vi "CSM-Logger-Thread.vi"(4 "Log Limit":T1={"file size (in bytes)"=10000000, "file num"=2} {"file size (in bytes)" format="%.0p"}, 6 "Exit When All Module Exist? (F)":bool, 7 "Format String":string="%<%Y/%m/%d %H:%M:%S%3u>T", 8 "error in (no error)":errorcluster, 9 "WatchDogQ":refnum<queue>, 10 "GlobalLogFilter.lvclass":refnum<class "LogFilter.lvclass">, 11 "File Path (Use Dialog)":path) -> (0 "error out":errorcluster)   [LabVIEW 2017, in "CSM File Logger.lvlib"]
doc: "The thread VI used in the CSM - Start File Logger VI.\n\n\n> [!NOTE] <b>CSM File Logger Implementation Principle</b>\n>\n> The CSM File Logger retrieves all execution records in the application via the CSM Global Log API and saves them to a specified text file for later analysis and error localization. The file format is a text file with the suffix `.csmlog`, which can be opened using text editing query tools such as Notepad."
uses:
  CSM File Logger.lvlib
  _Support/GlobalEvent/LogFilter/LogFilter.lvclass
  Communicable State Machine.lvlib
  _Support/Typedef/_CSM_List Module Scope.ctl
  _Shared/CSM Shared.lvlib
  CSM File Logger Limit.ctl
panel:
  in  "internal Stop":bool
  out "#MsgInQueue":i32
  out "size (in bytes)":i64
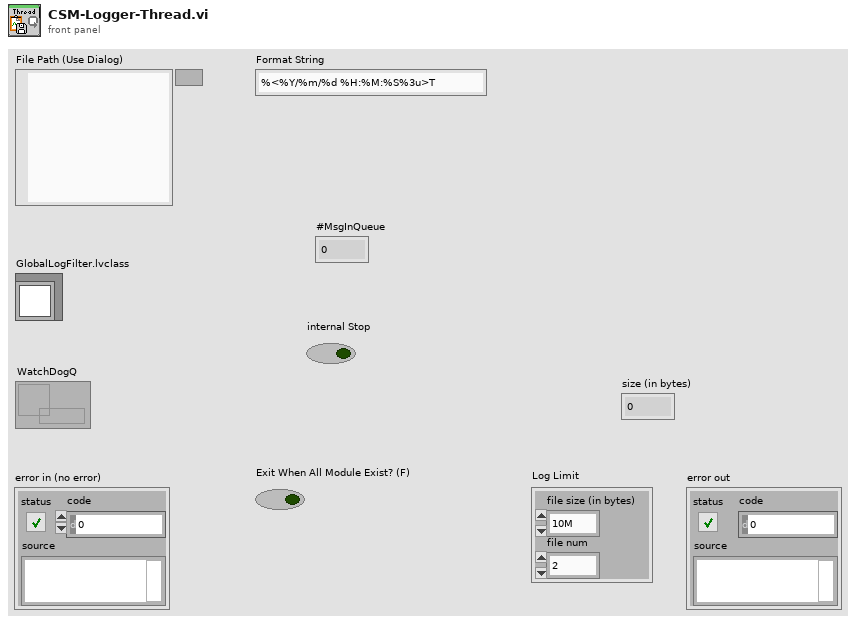
[diagram p1: front panel]
types:
  T1 = typedef "CSM File Logger.lvlib/CSM File Logger Limit.ctl" = cluster{"file size (in bytes)":i64, "file num":i32}
  T2 = typedef "Communicable State Machine.lvlib/_CSM_GlobalLog Filter Rules - v1.2.ctl" = cluster{"Global":cluster{"CSM":string[], "LogType":T3[], "State":string[], "StateType":T4[], "Broadcast":string[]}, "CSM":cluster{"LogType":cluster{"CSM":string, "LogType":T3}[], "State":cluster{"CSM":string, "State":string}[], "StateType":cluster{"CSM":string, "LogType":T4}[], "Broadcast":cluster{"CSM":string, "Broadcast":string}[]}, "PeriodicMessageFilter":cluster{"Enable":bool, "Threshold(#/s)":dbl, "CheckPeriod(s)":dbl}}
  T3 = typedef "Communicable State Machine.lvlib/_CSM_GlobalLog_MSG_TYPE.ctl" = enum16{"User Log", "State Change", "Status", "Interrupt", "Register", "Unregister", "Error Log", "Module Created", "Module Destroyed", "Async Message", "No-Rep Async Message", "Sync Message", "AsyncMsg Complete", "SyncMsg Complete"}
  T4 = typedef "Communicable State Machine.lvlib/_CSM_GlobalLog_STATE_TYPE.ctl" = enum16{"State - Internal State", "State - External Message", "State - Response", "State - Complete"}
  T5 = cluster{"Queue":path[], "folder":path, "name":string, "index":i32, "Log Limit":T1}
  T6 = enum16{"open", "replace", "create", "open or create", "replace or create", "replace or create with confirmation"}
  T7 = typedef "Communicable State Machine.lvlib/_CSM_List Module Scope.ctl" = enum16{"Normal", "System Only", "All"}
  T8 = typedef "Communicable State Machine.lvlib/Periodic String Filter Level.ctl" = enum16{"normal", "L1", "L2", "L3", "L4"}
  T9 = typedef "Communicable State Machine.lvlib/_CSM_GlobalLog_MSG.ctl" = cluster{"Name (\"\" to Use UUID)":string, "Current State":string, "Arguments":string, "Source Message":T10, "Source Module":string, "Complete(T)/Start(F)":bool, "LogType":T3, "Time Stamp":timestamp}
  T10 = typedef "Communicable State Machine.lvlib/_CSM_Response Source Message.ctl" = cluster{"‘State":string, "’Arguments":string, "’Error":errorcluster}
  T11 = cluster{"Major":u16, "Minor":u16, "Fix":u16, "Build":u16}
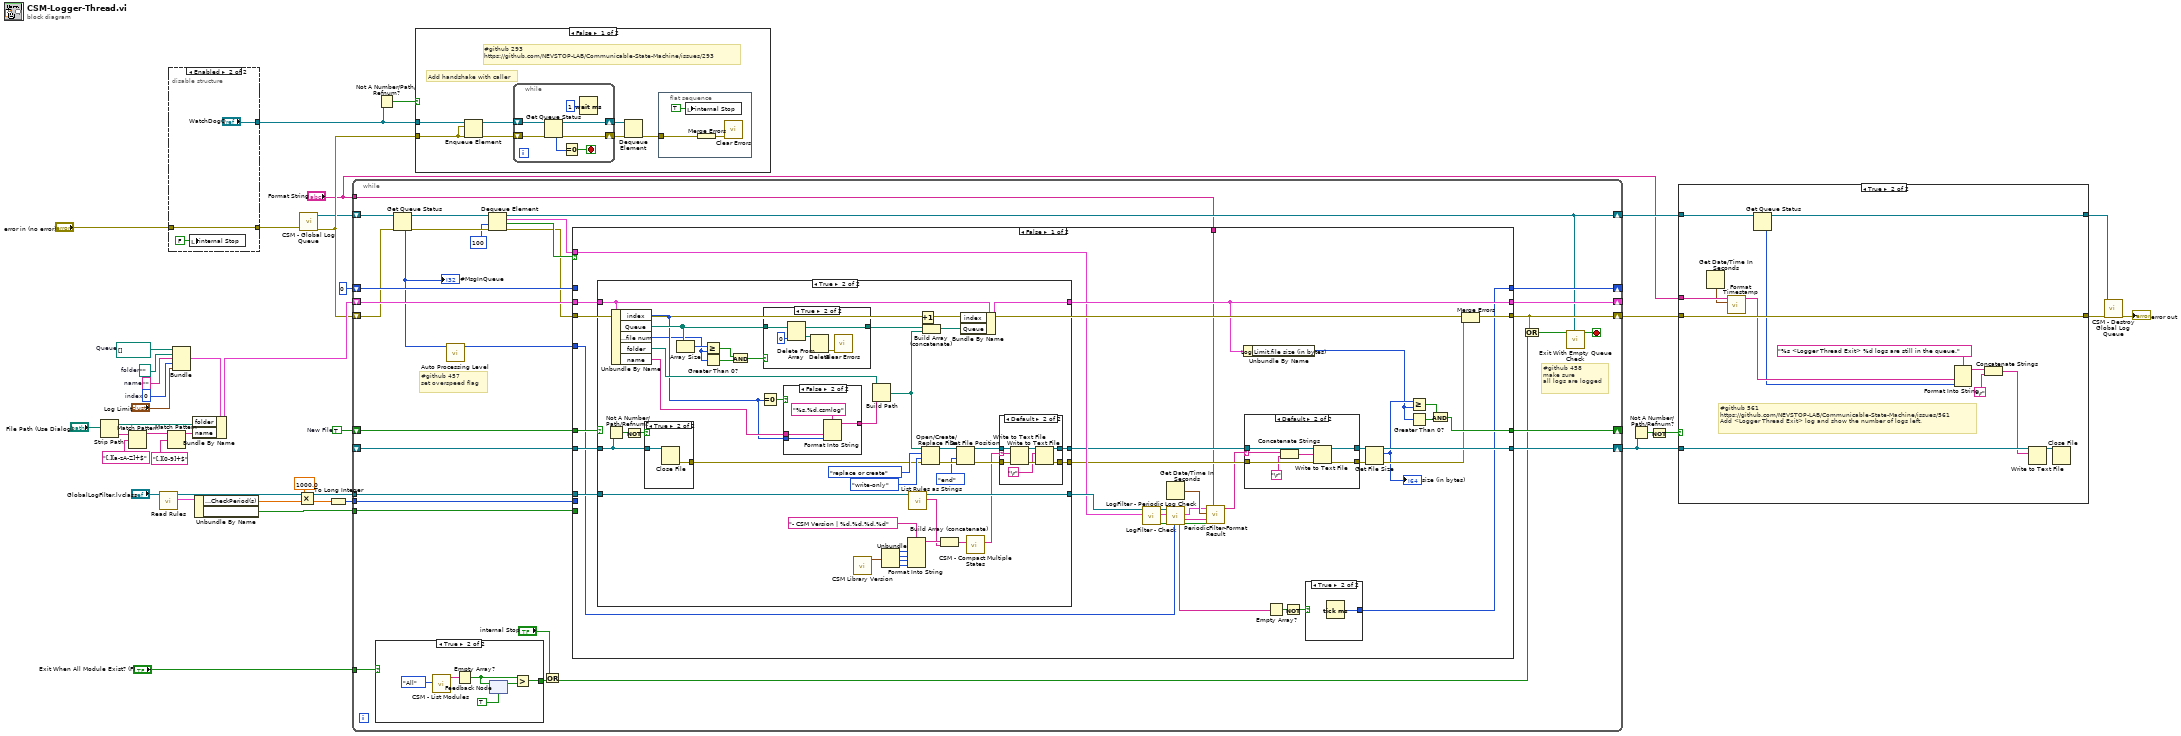
[diagram p0: block diagram]
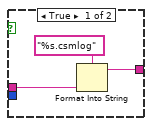
[diagram p6: hidden frame]
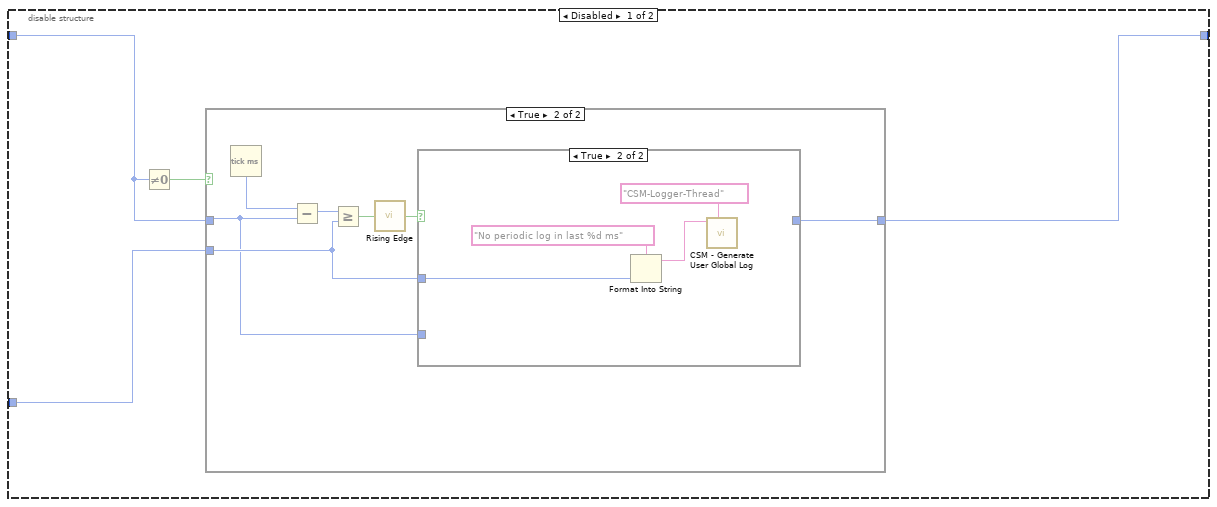
[diagram p10: hidden frame]
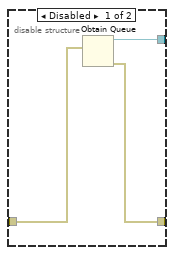
[diagram p15: hidden frame]
diagram:
  w28 = ""  # name
  w31 = 0  # index
  w32 = path ""  # folder
  w33 = path[] []  # Queue
  w34 = TRUE  # New File
  n1 = Strip Path(path="File Path (Use Dialog)") -> (stripped path=w21:path, name=w27:string)
  n2 = Match Pattern(string=w27, regular expression="[.][a-zA-Z]+$") -> (before substring=w24:string)  [unwired: 1 in, 3 out]
  n3 = call "Read Rules.vi"("LogFilter In"="GlobalLogFilter.lvclass") -> ("Rules"=w16:T2, "LogFilter Out"=w17:refnum<class "LogFilter.lvclass">)  [unwired: 8 in, 1 out]
  n4 = Match Pattern(string=w24, regular expression="[.][0-9]+$") -> (before substring=w22:string)  [unwired: 1 in, 3 out]
  n5 = disable-structure shown="Enabled" {
    disable-tunnel: [w41 "WatchDogQ"] -> w40
    disable-tunnel: [w43 w45] -> w6
    disable-tunnel: "error in (no error)" -> [w42 w45]
    frame Disabled {
      n6 = Obtain Queue(element data type=w42) -> (queue out=w41:refnum<queue>, error out=w43:errorcluster)  [unwired: 4 in, 1 out]
    }
    frame Enabled {
      n7 = local write "internal Stop"(FALSE ("internal Stop")) -> ()
    }
  }
  n8 = Bundle("Queue"=w33, "folder"=w32, "name"=w28, "index"=w31, "Log Limit"="Log Limit") -> (w29:T5)  [unwired: 1 in]
  n9 = Bundle By Name(cluster=w29, "folder"=w21, "name"=w22) -> (w23:T5)
  n10 = Unbundle By Name(w16) -> ("PeriodicMessageFilter.CheckPeriod(s)"=w14:dbl, "PeriodicMessageFilter.Enable"=w15:bool)
  n11 = Multiply(x=1000.0, y=w14) -> (x*y=w13:dbl)
  n12 = call "CSM - Global Log Queue.vi"("Error In"=w6) -> ("error out"=w9:errorcluster, "Global Log Queue"=w7:refnum<queue>)  [unwired: 9 in]
  n13 = To Long Integer(number=w13) -> (32bit integer=w11:i32)
  n14 = while {
    shift-right: [w76] -> w4
    shift-left: w9 -> [w59]
    shift-right: [w74] -> w36
    shift-left: _ -> [w75]
    tunnel: "Exit When All Module Exist? (F)" -> [w58]
    shift-right: [w72] -> _
    shift-left: w34 -> [w73]
    shift-right: [w70] -> _
    shift-left: w23 -> [w71]
    tunnel: w17 -> [w69]
    tunnel: w15 -> [w66]
    tunnel: w11 -> [w68]
    shift-right: [w67] -> _
    shift-left: u32 0 ("millisecond timer value") -> [w65]
    shift-right: [w50] -> w2
    shift-left: w7 -> [w62]
    tunnel: "Format String" -> [w47]
    stop <- w51 stop-if-true
    # "#github 458\nmake sure \nall logs are logged"
    # "#github 457\nset overspeed flag"
    n15 = case shown="True" w58 {
      tunnel: [_ w216] -> w57
      frame False {
      }
      frame True {
        n16 = call "CSM - List Modules.vi"("Scope (Normal)"=_CSM_List_Module_Scope."All" ("Mode")) -> ("Module Names"=w220:string[])  [unwired: 9 in, 1 out]
        n17 = Empty Array?(array=w220) -> (empty?=w219:bool)
        n18 = feedback #1(TRUE ("All?")) -> (w218:bool)
        n19 = feedback-in #1(w219) -> ()
        n20 = Greater?(x=w219, y=w218) -> (0:w216:bool)
      }
    }
    n21 = Get Queue Status(queue=w62, error in (no error)=w59) -> (queue out=w61:refnum<queue>, error out=w60:errorcluster, # elements in queue=w49:i32)  [unwired: 1 in, 5 out]
    "#MsgInQueue" <- w49
    n22 = call "Auto Processing Level.vi"("#Left In Q"=w49) -> ("Level"=w48:T8)  [unwired: 8 in, 2 out]
    n23 = Dequeue Element(queue=w61, timeout in ms (-1)=100, error in (no error)=w60) -> (queue out=w50:refnum<queue>, element=w53:T9, timed out?=w64:bool, error out=w63:errorcluster)
    n24 = Or(x="internal Stop", y=w57) -> (x .or. y?=w55:bool)
    n25 = case shown="False" w64 {
      tunnel: w63 -> [w110 w197]
      tunnel: [w109 w197] -> w76
      tunnel: w75 -> [w108 w196]
      tunnel: [w107 w196] -> w74
      tunnel: w73 -> [w106 w195]
      tunnel: [w105 w195] -> w72
      tunnel: w71 -> [w104 w194]
      tunnel: [w103 w194] -> w70
      tunnel: w69 -> [w102 _]
      tunnel: w68 -> [_ w193]
      tunnel: [w101 w191] -> w67
      tunnel: w66 -> [_ _]
      tunnel: w65 -> [_ w192]
      tunnel: w53 -> [w91 _]
      tunnel: w48 -> [w86 _]
      tunnel: w47 -> [w77 _]
      frame False {
        n26 = case shown="True" w106 {
          tunnel: w108 -> [w123 w163]
          tunnel: [_ w135] -> w88
          tunnel: [w123 w136] -> w87
          tunnel: [w122 w152] -> w103
          tunnel: w104 -> [w122 w154]
          tunnel: [w121 w134] -> w95
          tunnel: w102 -> [w121 w139]
          frame False {
          }
          frame True {
            n27 = Not A Number/Path/Refnum?(number/path/refnum=w163) -> (NaN/Path/Refnum?=w164:bool)
            n28 = Unbundle By Name(w154) -> ("index"=w144:i32, "Queue"=w155:path[], "Log Limit.file num"=w141:i32, "folder"=w148:path, "name"=w147:string)
            n29 = Not(x=w164) -> (.not. x?=w165:bool)
            n30 = case shown="True" w165 {
              tunnel: w163 -> [_ w190]
              tunnel: [_ w189] -> w157
              frame False {
              }
              frame True {
                n31 = Close File(refnum=w190) -> (error out=w189:errorcluster)  [unwired: 1 in, 1 out]
              }
            }
            n32 = Array Size(array=w155) -> (size(s)=w156:i32)
            n33 = Greater Or Equal?(x=w156, y=w141) -> (x >= y?=w143:bool)
            n34 = Greater Than 0?(x=w141) -> (x > 0?=w142:bool)
            n35 = And(x=w143, y=w142) -> (x .and. y?=w140:bool)
            n36 = Equal To 0?(x=w144) -> (x = 0?=w145:bool)
            n37 = case shown="True" w140 {
              tunnel: w155 -> [w183 w188]
              tunnel: [w183 w184] -> w153
              frame False {
              }
              frame True {
                n38 = Delete From Array(array=w188, index=0) -> (deleted portion=w186:path, array with subset deleted=w184:path[])  [unwired: 1 in]
                n39 = Delete(path (use dialog)=w186) -> (error out=w185:errorcluster)  [unwired: 4 in, 2 out]
                n40 = call <vilib>:"Clear Errors.vi"("error in (no error)"=w185) -> ()  [unwired: 5 in, 2 out]
              }
            }
            n41 = case shown="False" w145 {
              tunnel: [w177 w181] -> w149
              tunnel: w147 -> [w176 w180]
              tunnel: w144 -> [_ w179]
              frame True {
                n42 = Format Into String(format string="%s.csmlog", w176) -> (resulting string=w177:string)  [unwired: 2 in, 1 out]
              }
              frame False {
                n43 = Format Into String(format string="%s.%d.csmlog", w180, w179) -> (resulting string=w181:string)  [unwired: 2 in, 1 out]
              }
            }
            n44 = call "CSM Library Version.vi"() -> ("Min-Compatible Version"=w132:T11)  [unwired: 10 in, 1 out]
            n45 = Build Path(base path=w148, name or relative path=w149) -> (appended path=w146:path)
            n46 = Unbundle(w132) -> ("Major"=w128:u16, "Minor"=w129:u16, "Fix"=w130:u16, "Build"=w131:u16)
            n47 = Format Into String(format string="- CSM Version | %d.%d.%d.%d" ("String to Prepend to Source (\"\")"), w128, w129, w130, w131) -> (resulting string=w126:string)  [unwired: 2 in, 1 out]
            n48 = call "List Rules as Strings.vi"("GlobalLogFilter In"=w139) -> ("Rule Strings"=w125:string[], "GlobalLogFilter Out"=w134:refnum<class "LogFilter.lvclass">)  [unwired: 8 in, 1 out]
            n49 = Increment(x=w144) -> (x+1=w150:i32)
            n50 = Open/Create/Replace File(file path (use dialog)=w146, error in=w157, operation (0:open)=T6."replace or create", access (0:read/write)=enum16{"read/write", "read-only", "write-only"}."write-only") -> (refnum out=w162:refnum<file>, error out=w161:errorcluster)  [unwired: 2 in, 1 out]
            n51 = Build Array (concatenate)(w153, w146) -> (w151:path[])
            n52 = Build Array (concatenate)(w126, w125) -> (w124:string[])
            n53 = Set File Position(refnum=w162, from (0:start)=enum16{"start", "end", "current"}."end", error in=w161) -> (refnum out=w137:refnum<file>, error out=w138:errorcluster)  [unwired: 1 in]
            n54 = Bundle By Name(cluster=w154, "index"=w150, "Queue"=w151) -> (w152:T5)
            n55 = call "CSM - Compact Multiple States.vi"("Multiple States"=w124) -> ("States"=w133:string)  [unwired: 9 in]
            n56 = case shown="Default" w133 {
              selector: w133 -> [_ w175]
              tunnel: w138 -> [w166 w174]
              tunnel: w137 -> [w167 w173]
              tunnel: [w167 w170] -> w136
              tunnel: [w166 w169] -> w135
              frame "" {
              }
              frame Default {
                n57 = Write to Text File(file (use dialog)=w173, text=w175, error in=w174) -> (refnum out=w171:refnum<file>, error out=w172:errorcluster)  [unwired: 1 in, 1 out]
                n58 = Write to Text File(file (use dialog)=w171, text="\r", error in=w172) -> (refnum out=w170:refnum<file>, error out=w169:errorcluster)  [unwired: 1 in, 1 out]
              }
            }
          }
        }
        n59 = call "LogFilter - Check.vi"("Cross CSM Data In"=w91, "GlobalLogFilter In"=w95) -> ("Matched? (Dup)"=w82:bool, "Cross CSM Data Out"=w83:T9, "GlobalLogFilter.lvclass (Dup)"=w84:refnum<class "LogFilter.lvclass">)  [unwired: 7 in]
        n60 = Get Date/Time In Seconds() -> (seconds since 1Jan1904=w85:timestamp)
        n61 = call "LogFilter - Periodic Log Check.vi"("Level (Normal)"=w86, "Matched Previous?"=w82, "Cross CSM Data In"=w83, "GlobalLogFilter In"=w84) -> ("Matched? (Dup)"=w79:bool, "Additional Info"=w80:string[], "Cross CSM Data Out"=w81:T9, "Filtered Status"=w94:string[])  [unwired: 3 in, 1 out]
        n62 = call "PeriodicFilter-Format Result.vi"("Time Format String"=w77, "Filtered"=w79, "Additional Info"=w80, "Current Time"=w85, "Cross CSM Data In"=w81) -> ("States"=w78:string)  [unwired: 6 in]
        n63 = Unbundle By Name(w103) -> ("Log Limit.file size (in bytes)"=w96:i64)
        n64 = case shown="Default" w78 {
          selector: w78 -> [_ w114]
          tunnel: w88 -> [w111 w119]
          tunnel: w87 -> [w112 w118]
          tunnel: [w112 w117] -> w90
          tunnel: [w111 w116] -> w89
          frame "" {
          }
          frame Default {
            n65 = Concatenate Strings(w114, "\r") -> (w113:string)
            n66 = Write to Text File(file (use dialog)=w118, text=w113, error in=w119) -> (refnum out=w117:refnum<file>, error out=w116:errorcluster)  [unwired: 1 in, 1 out]
          }
        }
        n67 = Empty Array?(array=w94) -> (empty?=w93:bool)
        n68 = Not(x=w93) -> (.not. x?=w92:bool)
        n69 = case shown="True" w92 {
          tunnel: [_ w120] -> w101
          frame False {
          }
          frame True {
            n70 = Tick Count (ms)() -> (millisecond timer value=w120:u32)
          }
        }
        n71 = Get File Size(file=w90, error in=w89) -> (refnum out=w107:refnum<file>, size (in bytes)=w99:i64, 0:w100:errorcluster)
        "size (in bytes)" <- w99
        n72 = Greater Or Equal?(x=w99, y=w96) -> (x >= y?=w98:bool)
        n73 = Greater Than 0?(x=w96) -> (x > 0?=w97:bool)
        n74 = And(x=w98, y=w97) -> (x .and. y?=w105:bool)
        n75 = Merge Errors(w110, w100) -> (w109:errorcluster)
      }
      frame True {
        n76 = disable-structure shown="Enabled" {
          disable-tunnel: w193 -> [w201 _]
          disable-tunnel: w192 -> [w200 _]
          disable-tunnel: [w198 _] -> w191
          frame Disabled {
            n77 = Not Equal To 0?(x=w200) -> (x != 0?=w199:bool)
            n78 = case shown="True" w199 {
              tunnel: w200 -> [w202 w205]
              tunnel: w201 -> [_ w207]
              tunnel: [w202 w206] -> w198
              frame False {
              }
              frame True {
                n79 = Tick Count (ms)() -> (millisecond timer value=w209:u32)
                n80 = Subtract(x=w209, y=w205) -> (x-y=w208:u32)
                n81 = Greater Or Equal?(x=w208, y=w207) -> (x >= y?=w204:bool)
                n82 = call "Rising Edge.vi"("Signal"=w204) -> ("Rising Edge"=w203:bool)
                n83 = case shown="True" w203 {
                  tunnel: w207 -> [_ w211]
                  tunnel: [w210 _] -> w206
                  tunnel: w205 -> [w210 _]
                  frame False {
                  }
                  frame True {
                    n84 = Format Into String(format string="No periodic log in last %d ms" ("Log"), w211) -> (resulting string=w212:string)  [unwired: 2 in, 1 out]
                    n85 = call "CSM - Generate User Global Log.vi"("Place (\"\" to Use VI's Name)"="CSM-Logger-Thread" ("Place(\"\" to use VI's Name)"), "Log"=w212) -> ()  [unwired: 9 in, 1 out]
                  }
                }
              }
            }
          }
          frame Enabled {
          }
        }
      }
    }
    n86 = Or(x=w76, y=w55) -> (x .or. y?=w52:bool)
    n87 = call "Exit With Empty Queue Check.vi"("Queue"=w50, "Stop"=w52) -> ("Exit"=w51:bool)  [unwired: 8 in, 1 out]
  }
  n88 = Not A Number/Path/Refnum?(number/path/refnum=w40) -> (NaN/Path/Refnum?=w39:bool)
  n89 = case shown="False" w39 {
    tunnel: w40 -> [w226 _]
    tunnel: w9 -> [w221 _]
    frame False {
      # "#github 293 \nhttps://github.com/NEVSTOP-LAB/Communicable-State-Machine/issues/293"
      # "Add handshake with caller"
      n90 = Enqueue Element(queue=w226, element=w221, error in (no error)=w221) -> (queue out=w225:refnum<queue>, error out=w223:errorcluster)  [unwired: 1 in, 1 out]
      n91 = while {
        shift-right: [w233] -> w224
        shift-left: w225 -> [w234]
        shift-right: [w231] -> w222
        shift-left: w223 -> [w232]
        stop <- w229 stop-if-true
        n92 = Get Queue Status(queue=w234, error in (no error)=w232) -> (queue out=w233:refnum<queue>, error out=w231:errorcluster, # elements in queue=w230:i32)  [unwired: 1 in, 5 out]
        n93 = Equal To 0?(x=w230) -> (x = 0?=w229:bool)
        n94 = Wait (ms)(milliseconds to wait=u32 1) -> ()  [unwired: 1 out]
      }
      n95 = Dequeue Element(queue=w224, error in (no error)=w222) -> (error out=w227:errorcluster)  [unwired: 1 in, 3 out]
      n96 = flat-sequence {
        tunnel: w227 -> [w237]
        frame #0 {
          n97 = local write "internal Stop"(TRUE ("internal Stop")) -> ()
          n98 = Merge Errors(w237) -> (w236:errorcluster)
          n99 = call <vilib>:"Clear Errors.vi"("error in (no error)"=w236) -> ()  [unwired: 5 in, 2 out]
        }
      }
    }
    frame True {
    }
  }
  n100 = Not A Number/Path/Refnum?(number/path/refnum=w36) -> (NaN/Path/Refnum?=w37:bool)
  n101 = Not(x=w37) -> (.not. x?=w35:bool)
  n102 = case shown="True" w35 {
    tunnel: w36 -> [_ w252]
    tunnel: [w238 w250] -> w5
    tunnel: w4 -> [w238 w250]
    tunnel: [w239 w242] -> w3
    tunnel: w2 -> [w239 w249]
    tunnel: "Format String" -> [_ w246]
    frame False {
    }
    frame True {
      # "#github 561\nhttps://github.com/NEVSTOP-LAB/Communicable-State-Machine/issues/561\nAdd <Logger Thread Exit> log and show the number of logs left."
      n103 = Get Date/Time In Seconds() -> (seconds since 1Jan1904=w245:timestamp)
      n104 = call "Format Timestamp.vi"("Timestamp"=w245, "Format String"=w246) -> ("String"=w241:string)  [unwired: 9 in]
      n105 = Get Queue Status(queue=w249) -> (queue out=w242:refnum<queue>, # elements in queue=w240:i32)  [unwired: 2 in, 6 out]
      n106 = Format Into String(format string="%s <Logger Thread Exit> %d logs are still in the queue.", w241, w240) -> (resulting string=w243:string)  [unwired: 2 in, 1 out]
      n107 = Concatenate Strings(w243, "\r") -> (w247:string)
      n108 = Write to Text File(file (use dialog)=w252, text=w247) -> (refnum out=w251:refnum<file>)  [unwired: 2 in, 2 out]
      n109 = Close File(refnum=w251) -> ()  [unwired: 1 in, 2 out]
    }
  }
  n110 = call "CSM - Destroy Global Log Queue.vi"("Error In"=w5, "Global Log Queue"=w3) -> ("error out"=→"error out":errorcluster)  [unwired: 9 in]
